vi "Write Mouse Event Frame.vi"(11 "Replay Helper Loop In":T3) -> (3 "Replay Helper Loop Out":T3)   [LabVIEW 2026]
uses:
  User32.dll
  Replay.lvlib
  dependencies/src/global.vi
  dependencies/src/dependencies.lvlib
  dependencies/src/LUTVirtualKeySelector.ctl
  3d447ad9-a63f-4401-b3c5-38a1ebd2952b.vi
  <userlib>/_OpenG.lib/comparison/comparison.llb/openg_comparison__ogtk.lvlib
  6cc855f4-6c8e-465e-9ed0-3a173b85c1ed.vi
  <userlib>/_OpenG.lib/comparison/comparison.llb/U8 Changed__ogtk.vi
  dependencies/src/KeyboardLUTSelector.ctl
  Replay Helper Loop.ctl
  dependencies/src/KeyboardReplayKey.ctl
panel:
  out "Key":T1(ring)
  out "Virtual Key":T2=164
  out "value out":errorcluster
  out "x = 0?":bool
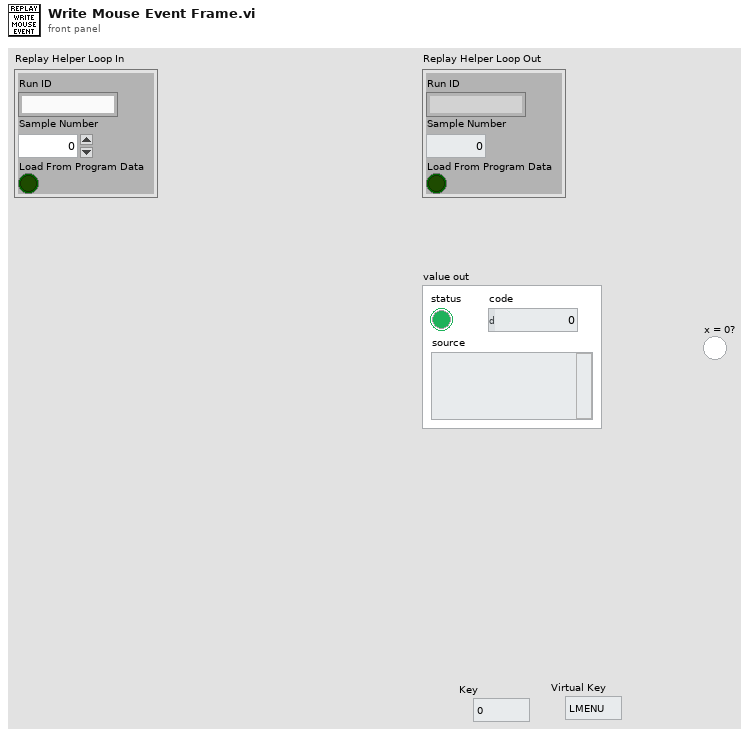
[diagram p1: front panel]
types:
  T1 = enum16{"0", "1", "2", "3", "4", "5", "6", "7", "8", "9", "A", "B", "C", "D", "E", "F", "G", "H", "I", "J", "K", "L", "M", "N", "O", "P", "Q", "R", "S", "T", "U", "V", "W", "X", "Y", "Z", "F1", "F2", "F3", "F4", "F5", "F6", "F7", "F8", "F9", "F10", "F11", "F12", "F13", "F14", "F15", "ADD", "BACK", "BACKSLASH", "CAPITAL", "COMMA", "DECIMAL", "DELETE", "DIVIDE", "DOWN", "END", "EQUALS", "ESCAPE", "GRAVE (`)", "HOME", "INSERT", "LBRACKET", "LCONTROL", "LEFT", "L ALT", "LSHIFT", "LWIN", "MINUS", "MULTIPLY", "NEXT", "NUMLOCK", "NUMPAD_0", "NUMPAD_1", "NUMPAD_2", "NUMPAD_3", "NUMPAD_4", "NUMPAD_5", "NUMPAD_6", "NUMPAD_7", "NUMPAD_8", "NUMPAD_9", "PAUSE", "PERIOD", "PRIOR (PG UP)", "RBRACKET", "RCONTROL", "RETURN", "RIGHT", "R ALT", "RSHIFT", "RWIN", "SCROLL", "SEMICOLON", "SLASH", "SPACE", "SUBTRACT", "TAB", "UP", "ENTER (num pad)", "' (quote)"}
  T2 = typedef "dependencies.lvlib/KeyboardReplayKey.ctl" = u8
  T3 = typedef "Replay.lvlib/Replay Helper Loop.ctl" = cluster{"Run ID":string, "Sample Number":i32, "Load From Program Data":bool}
  T4 = typedef "dependencies.lvlib/LUTVirtualKeySelector.ctl" = enum16{"Initialize", "Get Keyboard Event", "Set Keyboard Event"}
  T5 = typedef "dependencies.lvlib/KeyboardLUTSelector.ctl" = enum16{"Initialize", "Get Keyboards Keys Pressed at Sample Number", "Assign Keyboard Key Press to Sample Number"}
  T6 = typedef "dependencies.lvlib/KeyType.ctl" = enum16{"0", "1", "2", "3", "4", "5", "6", "7", "8", "9", "A", "B", "C", "D", "E", "F", "G", "H", "I", "J", "K", "L", "M", "N", "O", "P", "Q", "R", "S", "T", "U", "V", "W", "X", "Y", "Z", "F1", "F2", "F3", "F4", "F5", "F6", "F7", "F8", "F9", "F10", "F11", "F12", "F13", "F14", "F15", "ADD", "BACK", "BACKSLASH", "CAPITAL", "COMMA", "DECIMAL", "DELETE", "DIVIDE", "DOWN", "END", "EQUALS", "ESCAPE", "GRAVE (`)", "HOME", "INSERT", "LBRACKET", "LCONTROL", "LEFT", "L ALT", "LSHIFT", "LWIN", "MINUS", "MULTIPLY", "NEXT", "NUMLOCK", "NUMPAD_0", "NUMPAD_1", "NUMPAD_2", "NUMPAD_3", "NUMPAD_4", "NUMPAD_5", "NUMPAD_6", "NUMPAD_7", "NUMPAD_8", "NUMPAD_9", "PAUSE", "PERIOD", "PRIOR (PG UP)", "RBRACKET", "RCONTROL", "RETURN", "RIGHT", "R ALT", "RSHIFT", "RWIN", "SCROLL", "SEMICOLON", "SLASH", "SPACE", "SUBTRACT", "TAB", "UP", "ENTER (num pad)", "' (quote)"}
  T7 = cluster{"axis info":cluster{"Horizontal":i32, "Vertical":i32, "Scrolling":i32}, "button info":cluster{"button 1":bool, "button 2":bool, "button 3":bool, "button 4":bool}, "keyType":T6}
  T8 = cluster{"Horizontal":i32, "Vertical":i32, "Scrolling":i32}
  T9 = cluster{"button 1":bool, "button 2":bool, "button 3":bool, "button 4":bool}
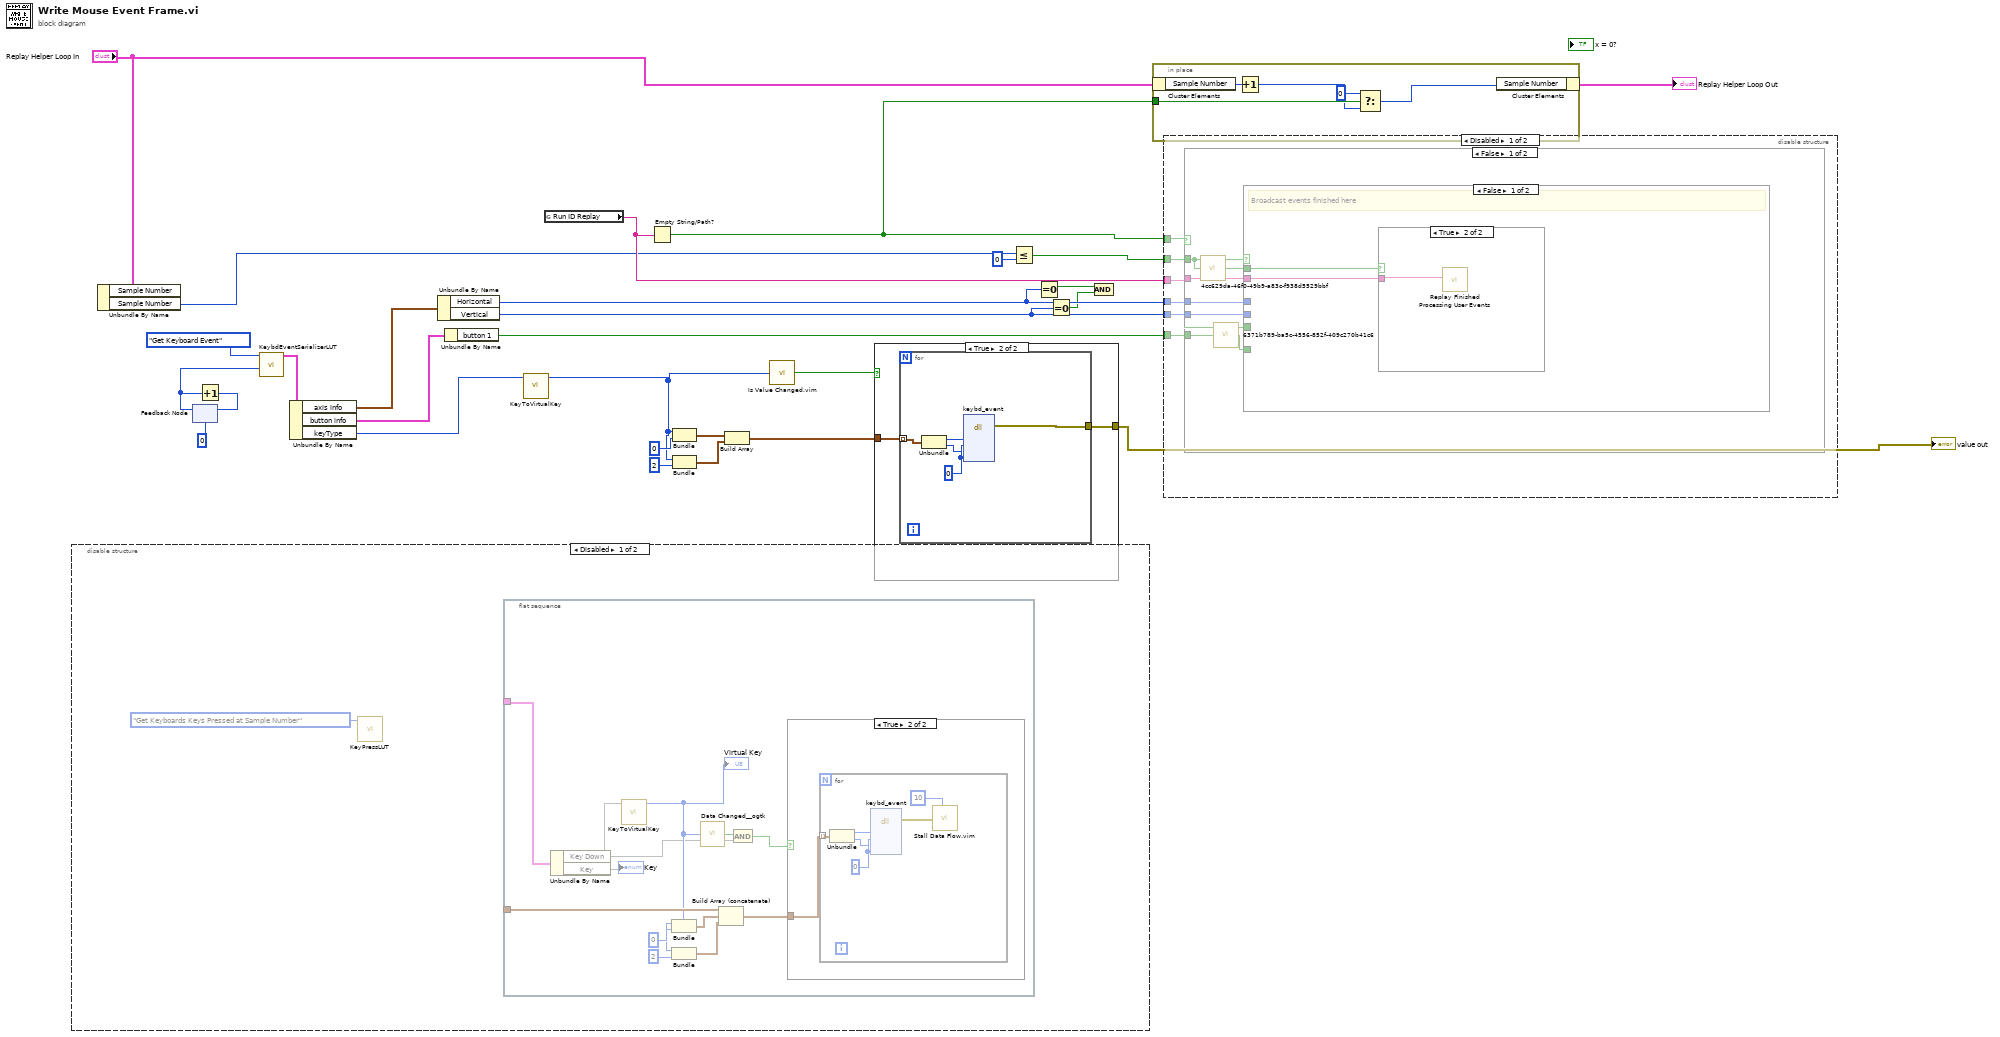
[diagram p0: block diagram]
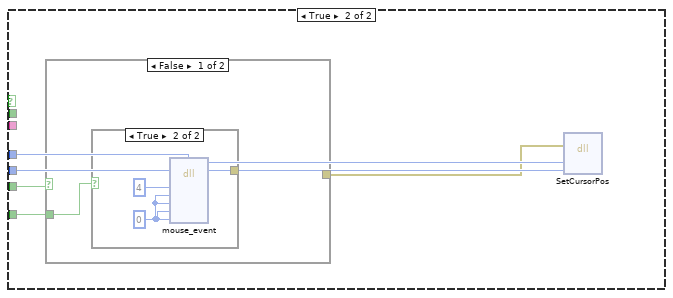
[diagram p3: hidden frame]
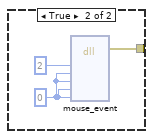
[diagram p6: hidden frame]
diagram:
  n1 = disable-structure shown="Disabled" {
    frame Disabled {
      n2 = call "KeyPressLUT.vi"("LUT Selector"=KeyboardLUTSelector."Get Keyboards Keys Pressed at Sample Number") -> ()  [unwired: 9 in, 2 out]
      n3 = flat-sequence {
        tunnel: _ -> [w41]
        tunnel: _ -> [w36]
        frame #0 {
          n4 = Unbundle By Name(w41) -> ("Key Down"=w31, "Key"=w40)
          "Key" <- w40
          n5 = call "KeyToVirtualKey.vi"("keyType Recorded"=w40) -> ("Virtual Key"=w33:T2)  [unwired: 9 in, 1 out]
          "Virtual Key" <- w33
          n6 = Bundle("Virtual Key"=w33, 0) -> (w38:cluster{"Virtual Key":T2, i32})  [unwired: 1 in]
          n7 = Bundle("Virtual Key"=w33, 2) -> (w39:cluster{"Virtual Key":T2, i32})  [unwired: 1 in]
          n8 = call-poly <userlib>:"Data Changed__ogtk.vi"("U8"=w33) -> ("Changed"=w32:bool)
          n9 = Build Array (concatenate)(w36, w38, w39) -> (w34:cluster{"Virtual Key":T2, i32}[])
          n10 = And(x=w32, y=w31) -> (x .and. y?=w30:bool)
          n11 = case shown="True" w30 {
            tunnel: w34 -> [_ w42]
            frame False {
            }
            frame True {
              n12 = for {
                tunnel: w42 -> [w47] mode=indexing
                w48 = u32 0 ("dwFlags")
                n13 = Unbundle(w47) -> ("Virtual Key"=w46:T2, w45:i32)
                n14 = dll-call lib="user32.dll" fn="keybd_event"("bVk"=w46, "bScan"=w48, "dwFlags"=w45, "dwExtraInfo"=w48) -> (error out=w44:errorcluster)  [unwired: 8 in, 1 out]
                n15 = call "Stall Data Flow.vim"("value in"=w44, "milliseconds to wait"=u32 10) -> ()  [unwired: 2 out]
              }
            }
          }
        }
      }
    }
    frame Enabled {
    }
  }
  n16 = Unbundle By Name("Replay Helper Loop In") -> ("Sample Number"=w19:i32)  [unwired: 1 out]
  n17 = feedback #1(u32 0 ("Iteration")) -> (w4:u32)
  n18 = Increment(x=w4) -> (x+1=w17:u32)
  n19 = feedback-in #1(w17) -> ()
  n20 = call "KeybdEventSerializerLUT.vi"("Iteration"=w4, "VirtualKeyLUTSelector"=LUTVirtualKeySelector."Get Keyboard Event") -> ("cluster"=w15:T7)  [unwired: 6 in, 3 out]
  n21 = Unbundle By Name(w15) -> ("axis info"=w14:T8, "button info"=w13:T9, "keyType"=w3:T6)
  n22 = Unbundle By Name(w14) -> ("Horizontal"=w28:i32, "Vertical"=w27:i32)
  n23 = Unbundle By Name(w13) -> ("button 1"=w12:bool)
  n24 = call "KeyToVirtualKey.vi"("keyType Recorded"=w3) -> ("Virtual Key"=w6:T2)  [unwired: 9 in, 1 out]
  n25 = global read "global.vi" "Run ID Replay"() -> (w23:string)
  n26 = Empty String/Path?(string/path=w23) -> (empty?=w20:bool)
  n27 = Bundle("Virtual Key"=w6, 0) -> (w10:cluster{"Virtual Key":T2, i32})  [unwired: 1 in]
  n28 = Bundle("Virtual Key"=w6, 2) -> (w8:cluster{"Virtual Key":T2, i32})  [unwired: 1 in]
  n29 = Build Array(w10, w8) -> (w7:cluster{"Virtual Key":T2, i32}[])
  n30 = call "Is Value Changed.vim"("value"=w6) -> ("changed or first call?"=w5:bool)
  n31 = case shown="True" w5 {
    tunnel: w7 -> [_ w50]
    tunnel: [_ w49] -> w2
    frame False {
    }
    frame True {
      n32 = for {
        tunnel: w50 -> [w52] mode=indexing
        tunnel: [w51] -> w49
        w55 = u32 0 ("dwFlags")
        n33 = Unbundle(w52) -> ("Virtual Key"=w54:T2, w53:i32)
        n34 = dll-call lib="user32.dll" fn="keybd_event"("bVk"=w54, "bScan"=w55, "dwFlags"=w53, "dwExtraInfo"=w55) -> (error out=w51:errorcluster)  [unwired: 8 in, 1 out]
      }
    }
  }
  "value out" <- w2
  n35 = Less Or Equal?(x=w19, y=0) -> (x <= y?=w24:bool)
  n36 = Equal To 0?(x=w28) -> (x = 0?=w26:bool)
  n37 = Equal To 0?(x=w27) -> (x = 0?=w25:bool)
  n38 = And(x=w26, y=w25) -> ()  [unwired: 1 out]
  n39 = in-place {
    in-place-border: w20 -> [w60]
    n40 = in-place-cluster #2("Replay Helper Loop In") -> ("Sample Number"=w59:i32)
    n41 = Increment(x=w59) -> (x+1=w58:i32)
    n42 = Select(t=0, s=w60, f=w58) -> (s? t:f=w57:i32)
    n43 = in-place-cluster #2("Sample Number"=w57) -> (→"Replay Helper Loop Out":T3)
  }
  n44 = disable-structure shown="Disabled" {
    disable-tunnel: w28 -> [w66 _]
    disable-tunnel: w27 -> [w65 _]
    disable-tunnel: w24 -> [w64 _]
    disable-tunnel: w23 -> [w63 _]
    disable-tunnel: w20 -> [w62 _]
    disable-tunnel: w12 -> [w61 _]
    frame Disabled {
      n45 = case shown="False" w62 {
        tunnel: w61 -> [w73 _]
        tunnel: w63 -> [w71 _]
        tunnel: w64 -> [w70 _]
        tunnel: w66 -> [w68 _]
        tunnel: w65 -> [w67 _]
        frame False {
          n46 = call "4cc629da-46f0-49b9-a83c-f938d5529bbf.vi"("value"=w70) -> ("changed or first call?"=w69:bool)
          n47 = call "6371b789-ba5c-4556-852f-409c270b41c6.vi"("value"=w73) -> ("changed or first call?"=w72:bool)
          n48 = case shown="False" w70 {
            tunnel: w68 -> [_ w81]
            tunnel: w67 -> [_ w80]
            tunnel: w73 -> [_ w79]
            tunnel: w72 -> [_ w78]
            tunnel: w71 -> [w74 _]
            tunnel: w69 -> [w75 _]
            frame False {
              # "Broadcast events finished here"
              n49 = case shown="True" w75 {
                tunnel: w74 -> [_ w76]
                frame False {
                }
                frame True {
                  n50 = call "Replay Finished Processing User Events.vi"("Run ID"=w76) -> ()  [unwired: 10 in, 1 out]
                }
              }
            }
            frame True {
              n51 = case shown="False" w79 {
                tunnel: w78 -> [w83 w88]
                tunnel: [w82 w87] -> w77
                frame False {
                  n52 = case shown="True" w83 {
                    tunnel: [_ w84] -> w82
                    frame False {
                    }
                    frame True {
                      w85 = u32 0 ("dy")
                      n53 = dll-call lib="user32.dll" fn="mouse_event"("dwFlags"=u32 4, "dx"=w85, "dy"=w85, "dwData"=w85, "dwExtraInfo"=w85) -> (error out=w84:errorcluster)  [unwired: 9 in, 1 out]
                    }
                  }
                }
                frame True {
                  n54 = case shown="False" w88 {
                    tunnel: [_ w89] -> w87
                    frame False {
                    }
                    frame True {
                      w90 = u32 0 ("dy")
                      n55 = dll-call lib="user32.dll" fn="mouse_event"("dwFlags"=u32 2, "dx"=w90, "dy"=w90, "dwData"=w90, "dwExtraInfo"=w90) -> (error out=w89:errorcluster)  [unwired: 9 in, 1 out]
                    }
                  }
                }
              }
              n56 = dll-call lib="User32.dll" fn="SetCursorPos" label="SetCursorPos (User32.dll)"(error in=w77, w81, w80) -> ()  [unwired: 4 in, 3 out]
            }
          }
        }
        frame True {
        }
      }
    }
    frame Enabled {
    }
  }
